vi "CE - OBW Marker Type.vi"(8 "error in (no error)":errorcluster, 11 "SA Measurement in":refnum<class "SA Measurement.lvclass">) -> (0 "error out":errorcluster, 3 "SA Measurement out":refnum<class "SA Measurement.lvclass">)   [LabVIEW 2023, in "Spectrum Analyzer.lvlib" / "SA Measurement.lvclass"]
uses:
  SA Measurement.lvclass
  Keysight 9020A/Keysight 9020A.lvclass
  D:/Project/IST013_CE Conduction Measurement/IST013-CE-Condcuted-Measurement/src/Spectrum Analyzer/Interface_Spectrum/Interface_Spectrum.lvclass
  TYPE DEFINITION/SA Measurement Class/TYPE CE OBW Setting Parameter.ctl
  TYPE DEFINITION/TYPE Y-axis Unit.ctl
  TYPE DEFINITION/TYPE Center and Span Frequency.ctl
  TYPE DEFINITION/TYPE Reference Level and Atten Param.ctl
  TYPE DEFINITION/TYPE Display Trace Mode Select.ctl
  TYPE DEFINITION/TYPE Detect Mode Select.ctl
  Keysight 9020A/Keysight 9020A.lvclass/Keysight 9020A.ctl
  SA Measurement.lvclass/SA Measurement.ctl
  Spectrum Analyzer.lvlib
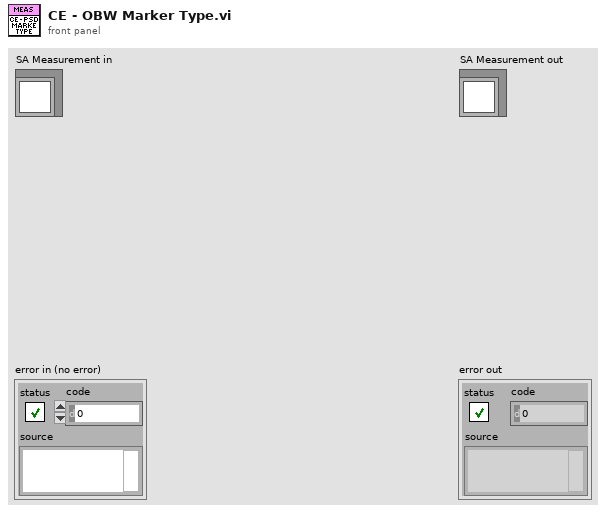
[diagram p1: front panel]
types:
  T1 = typedef "Spectrum Analyzer.lvlib/TYPE CE OBW Setting Parameter.ctl" = cluster{"Y-axis Unit":T2, "Center and Span Frequency(Hz)":T3, "Ref and Atten":T4, "Reference Offset":dbl, "External Preamp Gain":dbl, "RBW/VBW(Hz)":cluster{"RBW":dbl, "VBW":dbl}, "Sweep Time(s)":cluster{"Time":dbl, "Auto?":bool}, "OBW Setting":cluster{"BW Percent":dbl, "X dB":dbl, "Limit Frequency (Hz)":dbl, "Limit On?":bool, "Marker Position":enum16{"Left", "Right"}, "Marker On?":bool}, "Sweep Point":u32, "Avg/Hold Number":u32, "Trace and Detect":cluster{"Trace Mode":T5, "Detector Type":T6, "Detect Auto?":bool}[]}
  T2 = typedef "Spectrum Analyzer.lvlib/TYPE Y-axis Unit.ctl" = enum16{"dBm", "dBmV", "dBuV", "dBpW", "Volt", "Ampere", "Watt"}
  T3 = typedef "Spectrum Analyzer.lvlib/TYPE Center and Span Frequency.ctl" = cluster{"Center":dbl, "Span":dbl}
  T4 = typedef "Spectrum Analyzer.lvlib/TYPE Reference Level and Atten Param.ctl" = cluster{"Reference Level":dbl, "Atten":i32, "Atten Auto?":bool}
  T5 = typedef "Spectrum Analyzer.lvlib/TYPE Display Trace Mode Select.ctl" = enum16{"Clear Write", "Max Hold", "Min Hold", "Average", "View"}
  T6 = typedef "Spectrum Analyzer.lvlib/TYPE Detect Mode Select.ctl" = enum16{"Det Auto (Normal)", "Auto Peak", "Positive Peak", "Negative Peak", "Sample", "RMS", "Average", "Quasipeak", "CISPR Average", "RMS Average"}
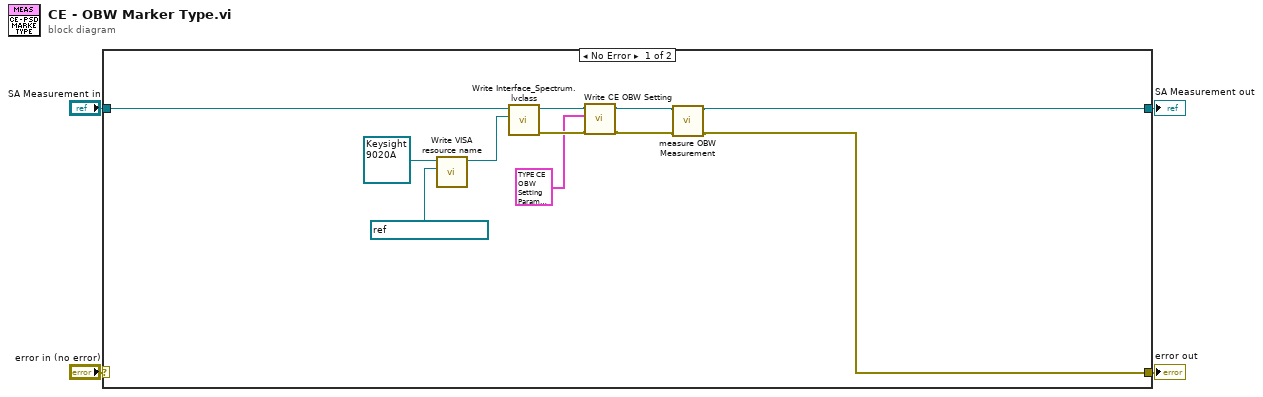
[diagram p0: block diagram]
diagram:
  n1 = case shown="No Error" "error in (no error)" {
    selector: "error in (no error)" -> [_ w17]
    tunnel: [w6 w17] -> w3
    tunnel: [w7 w16] -> w1
    tunnel: "SA Measurement in" -> [w13 w16]
    frame No Error {
      n2 = call "Write VISA resource name.vi"("VISA resource name"=refnum<visa-resource-name> "GPIB0::18::INSTR", "Keysight 9020A in"=refnum<class "Keysight 9020A.lvclass"> refnum ("Spectrum Analyzer.lvlib:Keysight 9020A.lvclass")) -> ("Keysight 9020A out"=w12:refnum<class "Keysight 9020A.lvclass">)  [unwired: 8 in, 1 out]
      n3 = call "Write Interface_Spectrum.lvclass.vi"("Interface_Spectrum.lvclass"=w12, "SA Measurement in"=w13) -> ("error out"=w10:errorcluster, "SA Measurement out"=w11:refnum<class "SA Measurement.lvclass">)  [unwired: 8 in]
      n4 = call "Write CE OBW Setting.vi"("error in (no error)"=w10, "Cluster"=T1 {"Y-axis Unit"=enum."dBm", "Center and Span Frequency(Hz)"={"Center"=2412000000.0, "Span"=40000000.0}, "Ref and Atten"={"Reference Level"=0.0, "Atten"=10, "Atten Auto?"=FALSE}, "Reference Offset"=0.0, "External Preamp Gain"=0.0, "RBW/VBW(Hz)"={"RBW"=300000.0, "VBW"=910000.0}, "Sweep Time(s)"={"Time"=1.0, "Auto?"=FALSE}, "OBW Setting"={"BW Percent"=99.0, "X dB"=-26.0, "Limit Frequency (Hz)"=20000000.0, "Limit On?"=TRUE, "Marker Position"=enum."Left", "Marker On?"=TRUE}, "Sweep Point"=1001, "Avg/Hold Number"=10, "Trace and Detect"=[{"Trace Mode"=enum."Max Hold", "Detector Type"=enum."Positive Peak", "Detect Auto?"=FALSE}]} ("CE OBW Setting"), "SA Measurement in"=w11) -> ("error out"=w8:errorcluster, "SA Measurement out"=w9:refnum<class "SA Measurement.lvclass">)  [unwired: 7 in]
      n5 = call "measure OBW Measurement.vi"("error in (no error)"=w8, "SA Measurement in"=w9) -> ("error out"=w6:errorcluster, "SA Measurement out"=w7:refnum<class "SA Measurement.lvclass">)  [unwired: 8 in]
    }
    frame Error {
    }
  }
  "error out" <- w3
  "SA Measurement out" <- w1
